vi "Dlg_Channel.vi"(0 "Channel":T1={"Name"="CH000", "Value"=0.0, "High Limit"=100.0, "Low Limit"=0.0, "Save"=TRUE, "Graph"=FALSE, "Scale Min"=0.0, "Scale Max"=100.0, "Unit"="%"}, 11 "error in":errorcluster) -> (4 "Channel out":T1={"Name"="CH000", "Value"=0.0, "High Limit"=100.0, "Low Limit"=0.0, "Save"=TRUE, "Graph"=FALSE, "Scale Min"=0.0, "Scale Max"=100.0, "Unit"="%"}, 6 "OK?":bool, 8 "Apply All":bool, 15 "error out":errorcluster)   [LabVIEW 2026]
doc: "채널 설정 팝업: 상한/하한, 저장(Save), 그래프(Graph), 스케일 Min/Max, 단위.\n'모든 채널에 적용'을 켜면 이름을 뺀 설정을 128채널 전체에 적용(Apply All)."
panel:
  in  "취소":bool
  in  "확인":bool
  in  "모든 채널에 적용":bool
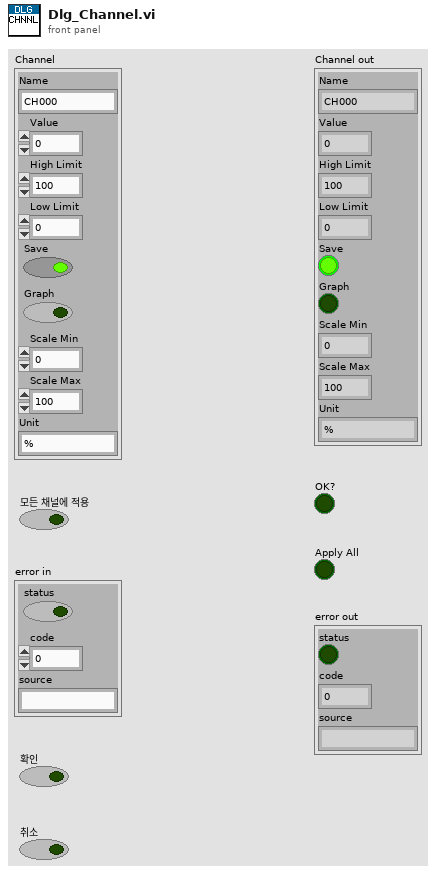
[diagram p1: front panel]
types:
  T1 = cluster{"Name":string, "Value":dbl, "High Limit":dbl, "Low Limit":dbl, "Save":bool, "Graph":bool, "Scale Min":dbl, "Scale Max":dbl, "Unit":string}
  T2 = cluster{"Left":i32, "Top":i32, "Right":i32, "Bottom":i32}
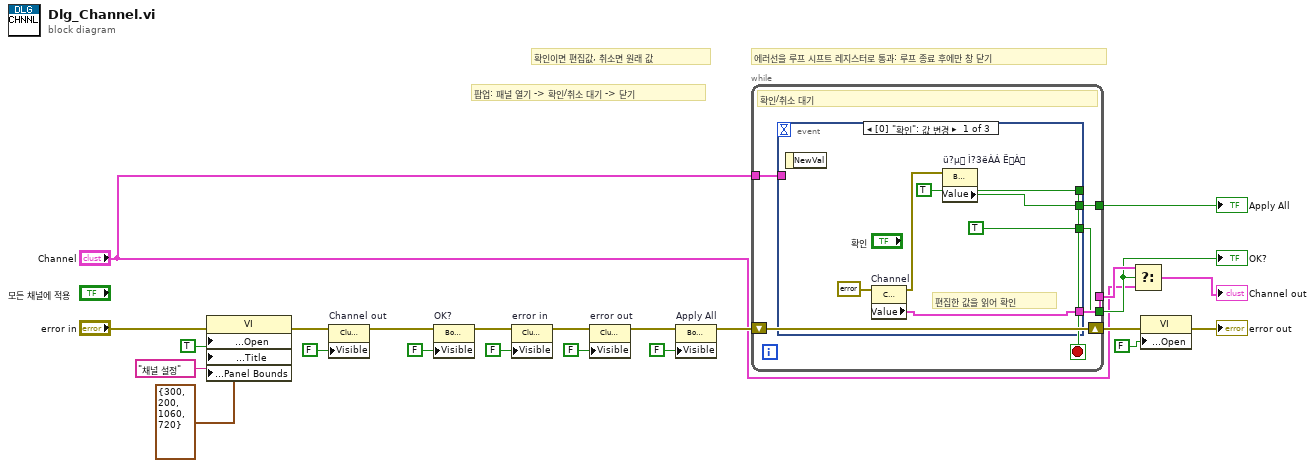
[diagram p0: block diagram]
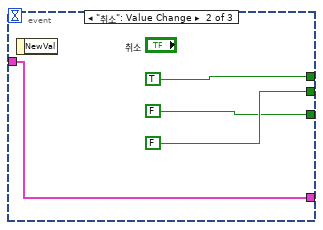
[diagram p2: hidden frame]
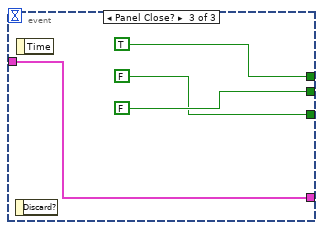
[diagram p3: hidden frame]
diagram:
  # "확인이면 편집값, 취소면 원래 값"
  # "에러선을 루프 시프트 레지스터로 통과: 루프 종료 후에만 창 닫기"
  # "팝업: 패널 열기 -> 확인/취소 대기 -> 닫기"
  n1 = property class="VI"(error in="error in", "Front Panel Window:Open"=TRUE, "Front Panel Window:Title"="채널 설정", "Front Panel Window:Panel Bounds"=T2 {"Left"=300, "Top"=200, "Right"=1060, "Bottom"=720}) -> (error out=w6:errorcluster)  [unwired: 1 in, 1 out]
  n2 = property on="Channel out" class="Clust (엄격한)"(error in=w6, "Visible"=FALSE) -> (error out=w8:errorcluster)  [unwired: 1 in, 1 out]
  n3 = property on="OK?" class="Bool (엄격한)"(error in=w8, "Visible"=FALSE) -> (error out=w10:errorcluster)  [unwired: 1 in, 1 out]
  n4 = property on="error in" class="Clust (엄격한)"(error in=w10, "Visible"=FALSE) -> (error out=w12:errorcluster)  [unwired: 1 in, 1 out]
  n5 = property on="error out" class="Clust (엄격한)"(error in=w12, "Visible"=FALSE) -> (error out=w14:errorcluster)  [unwired: 1 in, 1 out]
  n6 = property on="Apply All" class="Bool (엄격한)"(error in=w14, "Visible"=FALSE) -> (error out=w16:errorcluster)  [unwired: 1 in, 1 out]
  n7 = while {
    tunnel: "Channel" -> [w24]
    tunnel: [w26] -> w17
    tunnel: [w27] -> w18
    tunnel: [w28] -> w19
    shift-right: [w29] -> w20
    shift-left: w16 -> [w29]
    stop <- w25 stop-if-true
    # "확인/취소 대기"
    n8 = event shown="[0] \"확인\": 값 변경" {
      selector: _ -> [_ _ _]
      dyn-events: _ -> [_ _ _]
      timeout: _ -> [_ _ _]
      tunnel: [TRUE TRUE TRUE] -> w25
      tunnel: [TRUE FALSE FALSE] -> w26
      tunnel: w24 -> [_ w36 w40]
      tunnel: [w31 w36 w40] -> w27
      tunnel: [w35 FALSE FALSE] -> w28
      event "확인": Value Change {
        # "편집한 값을 읽어 확인"
        n9 = event-data() -> ()  [unwired: 1 in, 1 out]
        n10 = property on="Channel" class="Clust (엄격한)"(error in=errorcluster {"status"=FALSE, "code"=0, "source"=""}) -> (error out=w32:errorcluster, "Value"=w31:T1)  [unwired: 1 in, 1 out]
        n11 = property on="ü?µ Ì?3ëÀÁ ËÀ" class="Bool (엄격한)"(error in=w32) -> ("Value"=w35:bool)  [unwired: 1 in, 2 out]
      }
      event "취소": Value Change {
        n12 = event-data() -> ()  [unwired: 1 in, 1 out]
      }
      event Panel Close? {
        n13 = event-data() -> ()  [unwired: 2 in, 1 out]
        n14 = event-data() -> ()  [unwired: 1 in, 1 out]
      }
    }
  }
  "OK?" <- w17
  "Apply All" <- w19
  n15 = Select(t=w18, s=w17, f="Channel") -> (s? t:f=→"Channel out":T1)
  n16 = property class="VI"(error in=w20, "Front Panel Window:Open"=FALSE) -> (error out=→"error out":errorcluster)  [unwired: 1 in, 1 out]
